vi "probe-scale-by.vi"(0 "obj in":path, 1 "Factor":dbl=1.0) -> (2 "obj out":path)   [LabVIEW 2026]
doc: "Round14: Sensor's override of Can Scale:Scale By. Same pane shape as the interface declares (obj in, Factor, obj out); the diagram is a pass-through because a class-typed unbundle cannot be authored in AIXML."
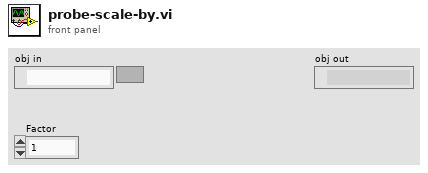
[diagram p1: front panel]
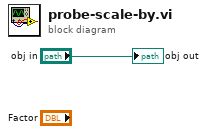
[diagram p0: block diagram]
diagram:
  "obj out" <- "obj in"
